vi "refresh Vbg.vi"(8 "stop":bool) -> (0 "X3":cluster{"Y":dbl[], "Y":dbl[]}[](graph), 1 "Zx 4":cluster{"Y":dbl[], "Y":dbl[]}[](graph), 2 "Zx 3":cluster{"Y":dbl[], "Y":dbl[]}[](graph), 3 "Temp vs Time":cluster{"Y":dbl[], "Y":dbl[]}[](graph), 4 "i X":cluster{"Y":dbl[], "Y":dbl[]}[](graph), 5 "X 2":cluster{"Y":dbl[], "Y":dbl[]}[](graph))   [LabVIEW 2011]
uses:
  DAQ-lockin-SubVI/Source/Lock-in Globles.vi
  SubVI/ITX_Global.vi
panel:
  in  "Tab Control":T1(tab)
  in  "Lock-in # 2":u16(ring)=1 items=["Lock-in #1", "Lock-in #2", "Lock-in #3", "Lock-in #4"]
  out "OSC Configuration":T2(array[cluster])=[{"Signal Type"=enum."Sine Wave", "DC"=0.0, "Amplitude"=0.15, "frequency"=1.3459999999999999, "Phase"=0.0}, {"Signal Type"=enum."Sine Wave", "DC"=0.0, "Amplitude"=0.0, "frequency"=1.346, "Phase"=0.0}, {"Signal Type"=enum."Sine Wave", "DC"=0.0, "Amplitude"=0.0, "frequency"=1.346, "Phase"=0.0}, {"Signal Type"=enum."Sine Wave", "DC"=0.0, "Amplitude"=0.0, "frequency"=1.346, "Phase"=0.0}] {"frequency" format="%0.2p"; "Amplitude" format="%0.2p"; "DC" format="%.2p"}
  in  "Lock-in # 1":u16(ring) items=["Lock-in #1", "Lock-in #2", "Lock-in #3", "Lock-in #4"]
  in  "Lock-in # 3":u16(ring)=2 items=["Lock-in #1", "Lock-in #2", "Lock-in #3", "Lock-in #4"]
  in  "Lock-in # 4":u16(ring)=3 items=["Lock-in #1", "Lock-in #2", "Lock-in #3", "Lock-in #4"]
  in  "milliseconds to wait":u32=1000
  in  "Comments":string="SA02628C 20120701\ncool down and warm up in ppms\n2 terminal tests.\nI+/I- : 3/27\nV+V-: 1/28\n\n\n\nno back gate voltage connected\n"
  out "Connected":string="I+:2\nV1+:3\nI-:28\nV-:5\n"
  in  "Vbg interval":u32=3000
  in  "Vo":dbl=-2.0
  in  "Vmax":dbl=7.0
  out "Vbg":dbl=-2.0
  in  "dV":dbl=0.01
  in  "Vmin":dbl=-2.0
  in  "OK Button":bool
  in  "Vsg     Vbg":bool
  in  "OSC config channel#":i32
  in  "Vsg interval":u32=3000
  out "Vsg":dbl
  out "Vbg vs time":cluster{"Y":dbl[], "Y":dbl[]}[](graph)
  out "Vsg vs time":cluster{"Y":dbl[], "Y":dbl[]}[](graph)
  out "i Y":cluster{"Y":dbl[], "Y":dbl[]}[](graph)
  out "i X 3":cluster{"Y":dbl[], "Y":dbl[]}[](graph)
  out "i Y 3":cluster{"Y":dbl[], "Y":dbl[]}[](graph)
  out "Y 2":cluster{"Y":dbl[], "Y":dbl[]}[](graph)
  out "Y3":cluster{"Y":dbl[], "Y":dbl[]}[](graph)
  out "Zy 3":cluster{"Y":dbl[], "Y":dbl[]}[](graph)
  out "Zy 4":cluster{"Y":dbl[], "Y":dbl[]}[](graph)
  out "i X 2":cluster{"Y":dbl[], "Y":dbl[]}[](graph)
  out "i X 4":cluster{"Y":dbl[], "Y":dbl[]}[](graph)
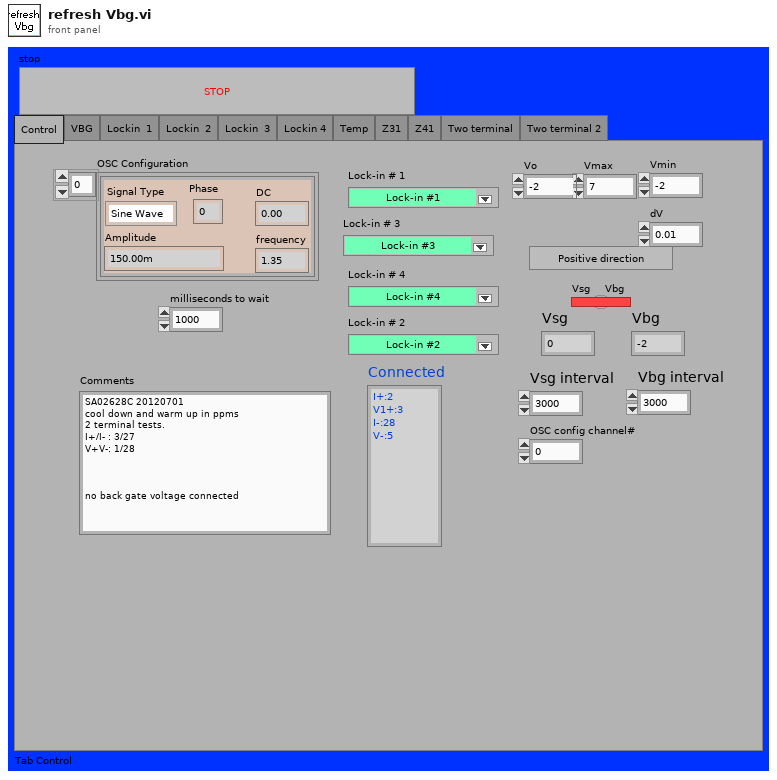
[diagram p1: front panel]
types:
  T1 = enum32{"Control", "VBG", "Lockin  1", "Lockin  2", "Lockin  3", "Lockin 4", "Temp", "Z31", "Z41", "Two terminal", "Two terminal 2"}
  T2 = cluster{"Signal Type":enum16{"Sine Wave", "Triangle Wave", "Square Wave", "Sawtooth Wave"}, "DC":dbl, "Amplitude":dbl, "frequency":dbl, "Phase":dbl}[]
  T3 = cluster{"Signal Type":enum16{"Sine Wave", "Triangle Wave", "Square Wave", "Sawtooth Wave"}, "DC":dbl, "Amplitude":dbl, "frequency":dbl, "Phase":dbl}
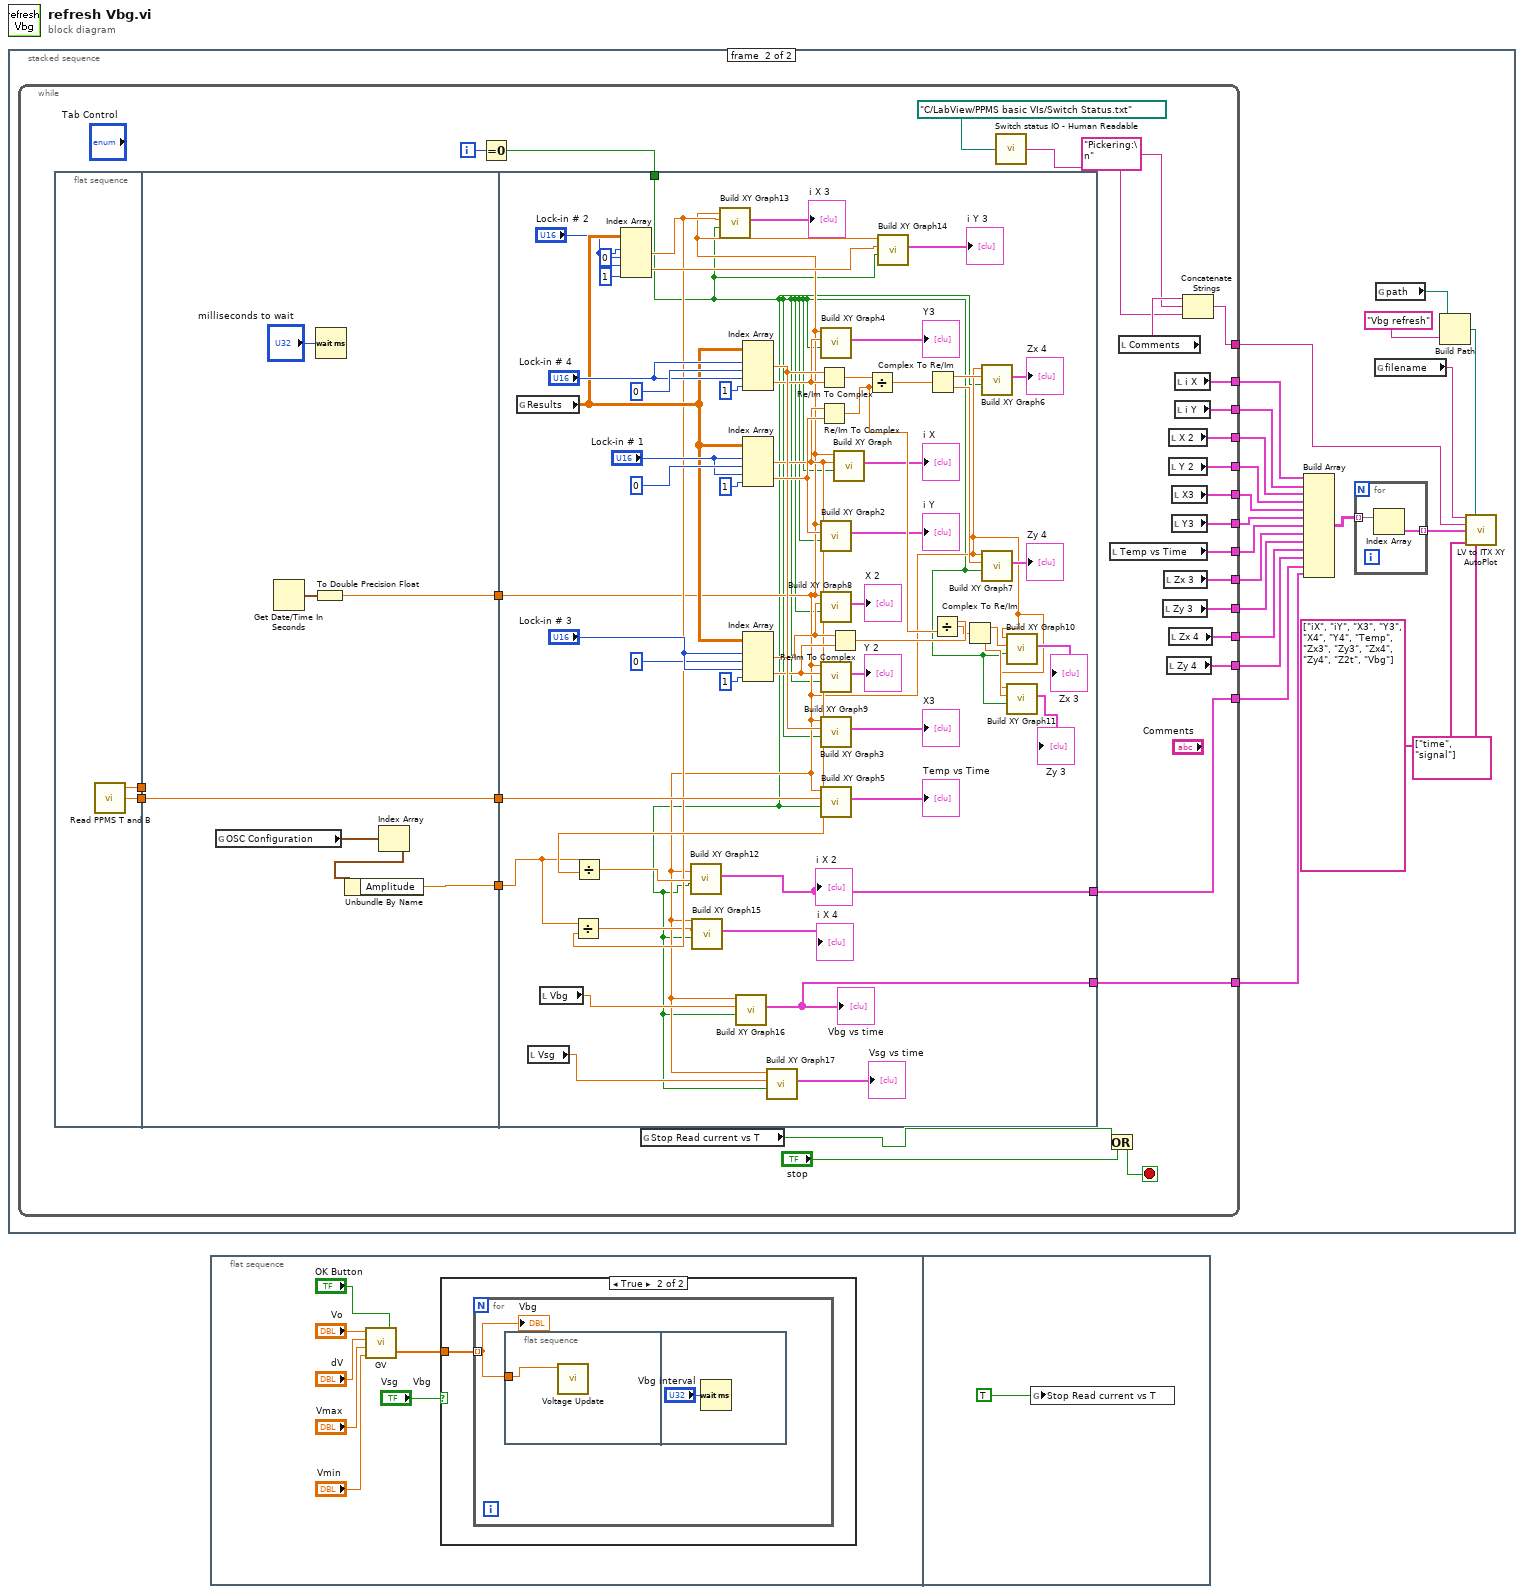
[diagram p0: block diagram]
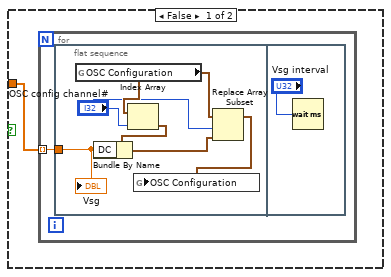
[diagram p2: hidden frame]
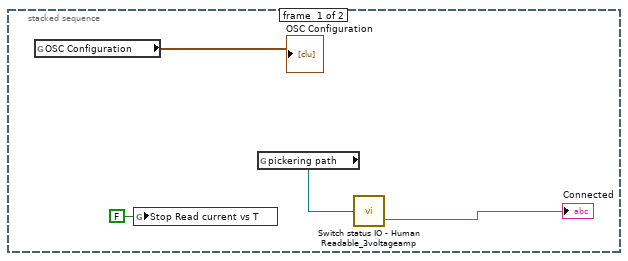
[diagram p3: hidden frame]
diagram:
  n1 = stacked-sequence {
    frame #0 {
      n2 = global read "Lock-in Globles.vi" "OSC Configuration"() -> (→"OSC Configuration":T2)
      n3 = global write "Lock-in Globles.vi" "Stop Read current vs T"(FALSE ("Stop Read current vs T")) -> ()
      n4 = global read "ITX_Global.vi" "pickering path"() -> (w1:path)
      n5 = call <userlib>:"Switch status IO - Human Readable_3voltageamp.vi"("Switch status"=w1) -> ("String"=→"Connected":string)  [unwired: 3 in]
    }
    frame #1 {
      n6 = while {
        tunnel: [w48] -> w26
        tunnel: [w47] -> w25
        tunnel: [w46] -> w24
        tunnel: [w45] -> w23
        tunnel: [w44] -> w22
        tunnel: [w43] -> w21
        tunnel: [w42] -> w20
        tunnel: [w41] -> w19
        tunnel: [w40] -> w18
        tunnel: [w39] -> w17
        tunnel: [w38] -> w16
        tunnel: [w36] -> w12
        tunnel: [w30] -> w6
        tunnel: [w29] -> w5
        i -> [w54]
        stop <- w50 stop-if-true
        n7 = flat-sequence {
          tunnel: [w58] -> w55
          tunnel: [w57] -> w51
          tunnel: [w64] -> w56
          tunnel: w55 -> [w64]
          tunnel: [w62] -> w52
          tunnel: w51 -> [_]
          tunnel: [w59] -> w31
          tunnel: w56 -> [w102]
          tunnel: w53 -> [w66]
          tunnel: w52 -> [w67]
          tunnel: w31 -> [w75]
          tunnel: [w83] -> w30
          tunnel: [w70] -> w29
          frame #0 {
            n8 = call "Read PPMS T and B.vi"() -> ("Temperature"=w58:dbl, "Time"=w57:dbl)  [unwired: 3 in, 1 out]
          }
          frame #1 {
            n9 = global read "Lock-in Globles.vi" "OSC Configuration"() -> (w61:T2)
            n10 = Get Date/Time In Seconds() -> (seconds since 1Jan1904=w63:timestamp)
            n11 = To Double Precision Float(number=w63) -> (double precision float=w62:dbl)
            n12 = Wait (ms)(milliseconds to wait="milliseconds to wait") -> ()  [unwired: 1 out]
            n13 = Index Array(array=w61) -> (element=w60:T3)  [unwired: 1 in]
            n14 = Unbundle By Name(w60) -> ("Amplitude"=w59:dbl)
          }
          frame #2 {
            n15 = global read "Lock-in Globles.vi" "Results"() -> (w82:dbl[][])
            n16 = local read "Vsg"() -> (w68:dbl)
            n17 = local read "Vbg"() -> (w71:dbl)
            n18 = Index Array(array=w82, index (row) #1="Lock-in # 2", index (col) #1=0 ("disabled index (col)"), index (row) #2="Lock-in # 2", index (col) #2=1 ("disabled index (col)")) -> (element #1=w74:dbl, element #2=w76:dbl)
            n19 = Divide(x=w75, y=w74) -> (x/y=w73:dbl)
            n20 = call "Build XY Graph15"("Reset"=w66, "Y Input"=w73, "X Input"=w67) -> ("XY Graph"=→"i X 4":cluster{"Y":dbl[], "Y":dbl[]}[])  [unwired: 2 in, 6 out]
            n21 = call "Build XY Graph13"("Reset"=w66, "Y Input"=w74, "X Input"=w67) -> ("XY Graph"=→"i X 3":cluster{"Y":dbl[], "Y":dbl[]}[])  [unwired: 2 in, 6 out]
            n22 = call "Build XY Graph16"("Reset"=w66, "Y Input"=w71, "X Input"=w67) -> ("XY Graph"=w70:cluster{"Y":dbl[], "Y":dbl[]}[])  [unwired: 2 in, 6 out]
            "Vbg vs time" <- w70
            n23 = Index Array(array=w82, index (row) #1="Lock-in # 4", index (col) #1=0 ("disabled index (col)"), index (row) #2="Lock-in # 4", index (col) #2=1 ("disabled index (col)")) -> (element #1=w110:dbl, element #2=w109:dbl)
            n24 = Index Array(array=w82, index (row) #1="Lock-in # 1", index (col) #1=0 ("disabled index (col)"), index (row) #2="Lock-in # 1", index (col) #2=1 ("disabled index (col)")) -> (element #1=w85:dbl, element #2=w111:dbl)
            n25 = Divide(x=w75, y=w85) -> (x/y=w84:dbl)
            n26 = call "Build XY Graph12"("Reset"=w66, "Y Input"=w84, "X Input"=w67) -> ("XY Graph"=w83:cluster{"Y":dbl[], "Y":dbl[]}[])  [unwired: 2 in, 6 out]
            "i X 2" <- w83
            n27 = Index Array(array=w82, index (row) #1="Lock-in # 3", index (col) #1=0 ("disabled index (col)"), index (row) #2="Lock-in # 3", index (col) #2=1 ("disabled index (col)")) -> (element #1=w96:dbl, element #2=w95:dbl)
            n28 = call "Build XY Graph17"("Reset"=w66, "Y Input"=w68, "X Input"=w67) -> ("XY Graph"=→"Vsg vs time":cluster{"Y":dbl[], "Y":dbl[]}[])  [unwired: 2 in, 6 out]
            n29 = Re/Im To Complex(1:w109, 2:w110) -> (0:w108:cdb)
            n30 = Re/Im To Complex(1:w111, 2:w85) -> (0:w93:cdb)
            n31 = call "Build XY Graph4"("Reset"=w66, "Y Input"=w109, "X Input"=w67) -> ("XY Graph"=→"Y3":cluster{"Y":dbl[], "Y":dbl[]}[])  [unwired: 2 in, 6 out]
            n32 = call "Build XY Graph2"("Reset"=w66, "Y Input"=w111, "X Input"=w67) -> ("XY Graph"=→"i Y":cluster{"Y":dbl[], "Y":dbl[]}[])  [unwired: 2 in, 6 out]
            n33 = call "Build XY Graph8"("Reset"=w66, "Y Input"=w96, "X Input"=w67) -> ("XY Graph"=→"X 2":cluster{"Y":dbl[], "Y":dbl[]}[])  [unwired: 2 in, 6 out]
            n34 = call "Build XY Graph9"("Reset"=w66, "Y Input"=w95, "X Input"=w67) -> ("XY Graph"=→"Y 2":cluster{"Y":dbl[], "Y":dbl[]}[])  [unwired: 2 in, 6 out]
            n35 = call "Build XY Graph3"("Reset"=w66, "Y Input"=w110, "X Input"=w67) -> ("XY Graph"=→"X3":cluster{"Y":dbl[], "Y":dbl[]}[])  [unwired: 2 in, 6 out]
            n36 = call "Build XY Graph5"("Reset"=w66, "Y Input"=w102, "X Input"=w67) -> ("XY Graph"=→"Temp vs Time":cluster{"Y":dbl[], "Y":dbl[]}[])  [unwired: 2 in, 6 out]
            n37 = Re/Im To Complex(1:w95, 2:w96) -> (0:w94:cdb)
            n38 = call "Build XY Graph"("Reset"=w66, "Y Input"=w85, "X Input"=w67) -> ("XY Graph"=→"i X":cluster{"Y":dbl[], "Y":dbl[]}[])  [unwired: 2 in, 6 out]
            n39 = Divide(x=w108, y=w93) -> (x/y=w107:cdb)
            n40 = call "Build XY Graph14"("Reset"=w66, "Y Input"=w76, "X Input"=w67) -> ("XY Graph"=→"i Y 3":cluster{"Y":dbl[], "Y":dbl[]}[])  [unwired: 2 in, 6 out]
            n41 = Complex To Re/Im(x + iy=w107) -> (x=w105:dbl, y=w106:dbl)
            n42 = Divide(x=w94, y=w93) -> (x/y=w92:cdb)
            n43 = Complex To Re/Im(x + iy=w92) -> (x=w91:dbl, y=w90:dbl)
            n44 = call "Build XY Graph6"("Reset"=w66, "Y Input"=w105, "X Input"=w67) -> ("XY Graph"=→"Zx 4":cluster{"Y":dbl[], "Y":dbl[]}[])  [unwired: 2 in, 6 out]
            n45 = call "Build XY Graph7"("Reset"=w66, "Y Input"=w106, "X Input"=w67) -> ("XY Graph"=→"Zy 4":cluster{"Y":dbl[], "Y":dbl[]}[])  [unwired: 2 in, 6 out]
            n46 = call "Build XY Graph10"("Reset"=w66, "Y Input"=w91, "X Input"=w67) -> ("XY Graph"=→"Zx 3":cluster{"Y":dbl[], "Y":dbl[]}[])  [unwired: 2 in, 6 out]
            n47 = call "Build XY Graph11"("Reset"=w66, "Y Input"=w90, "X Input"=w67) -> ("XY Graph"=→"Zy 3":cluster{"Y":dbl[], "Y":dbl[]}[])  [unwired: 2 in, 6 out]
          }
        }
        n48 = Equal To 0?(x=w54) -> (x = 0?=w53:bool)
        n49 = global read "Lock-in Globles.vi" "Stop Read current vs T"() -> (w32:bool)
        n50 = call <userlib>:"Switch status IO - Human Readable.vi"("Switch status"=path "C:/LabView/PPMS basic VIs/Switch Status.txt") -> ("String"=w33:string)
        n51 = Or(x=w32, y="stop") -> (x .or. y?=w50:bool)
        n52 = local read "Temp vs Time"() -> (w42:cluster{"Y":dbl[], "Y":dbl[]}[])
        n53 = local read "Comments"() -> (w35:string)
        n54 = local read "Zy 3"() -> (w40:cluster{"Y":dbl[], "Y":dbl[]}[])
        n55 = local read "Zx 3"() -> (w41:cluster{"Y":dbl[], "Y":dbl[]}[])
        n56 = local read "Zy 4"() -> (w38:cluster{"Y":dbl[], "Y":dbl[]}[])
        n57 = local read "X 2"() -> (w46:cluster{"Y":dbl[], "Y":dbl[]}[])
        n58 = local read "Y 2"() -> (w45:cluster{"Y":dbl[], "Y":dbl[]}[])
        n59 = local read "Zx 4"() -> (w39:cluster{"Y":dbl[], "Y":dbl[]}[])
        n60 = local read "X3"() -> (w44:cluster{"Y":dbl[], "Y":dbl[]}[])
        n61 = local read "Y3"() -> (w43:cluster{"Y":dbl[], "Y":dbl[]}[])
        n62 = local read "i X"() -> (w48:cluster{"Y":dbl[], "Y":dbl[]}[])
        n63 = local read "i Y"() -> (w47:cluster{"Y":dbl[], "Y":dbl[]}[])
        n64 = Concatenate Strings(w35, "Pickering:\n" ("string"), w33) -> (w36:string)
      }
      n65 = Build Array(w26, w25, w24, w23, w22, w21, w20, w19, w18, w17, w16, w6, w5) -> (w15:cluster{"Y":dbl[], "Y":dbl[]}[][])
      n66 = for {
        tunnel: w15 -> [w28] mode=indexing
        tunnel: [w27] -> w14 mode=indexing
        n67 = Index Array(array=w28) -> (element=w27:cluster{"Y":dbl[], "Y":dbl[]})  [unwired: 1 in]
      }
      n68 = global read "ITX_Global.vi" "filename"() -> (w13:string)
      n69 = global read "ITX_Global.vi" "path"() -> (w9:path)
      n70 = Build Path(base path=w9, name or relative path="Vbg refresh") -> (appended path=w8:path)
      n71 = call <userlib>:"LV to ITX XY AutoPlot.vi"("filename"=w13, "path"=w8, "Notes"=w12, "XY Array"=w14, "wavenames (.Vx, etc)"=string[] ["iX", "iY", "X3", "Y3", "X4", "Y4", "Temp", "Zx3", "Zy3", "Zx4", "Zy4", "Z2t", "Vbg"], "X,Y Labels"=string[] ["time", "signal"]) -> ()  [unwired: 9 in, 1 out]
    }
  }
  n72 = flat-sequence {
    frame #0 {
      n73 = call "GV.vi"("OK Button"="OK Button", "Vmin"="Vmin", "Vmax"="Vmax", "dV"="dV", "Vo"="Vo") -> ("Waveform Graph"=w122:dbl[])
      n74 = case shown="True" "Vsg     Vbg" {
        tunnel: w122 -> [w128 w137]
        frame False {
          n75 = for {
            tunnel: w128 -> [w129] mode=indexing
            n76 = flat-sequence {
              tunnel: w129 -> [w130]
              frame #0 {
                n77 = global read "Lock-in Globles.vi" "OSC Configuration"() -> (w134:T2)
                n78 = Index Array(array=w134, index="OSC config channel#") -> (element=w135:T3)
                n79 = Bundle By Name(cluster=w135, "DC"=w130) -> (w132:T3)
                n80 = Replace Array Subset(array=w134, new element=w132, index="OSC config channel#") -> (w131:T2)
                n81 = global write "Lock-in Globles.vi" "OSC Configuration"(w131) -> ()
                "Vsg" <- w130
              }
              frame #1 {
                n82 = Wait (ms)(milliseconds to wait="Vsg interval") -> ()  [unwired: 1 out]
              }
            }
          }
        }
        frame True {
          n83 = for {
            tunnel: w137 -> [w138] mode=indexing
            n84 = flat-sequence {
              tunnel: w138 -> [w139]
              frame #0 {
                n85 = call "Voltage Update.vi"("Voltage Output"=w139) -> ()  [unwired: 8 in]
              }
              frame #1 {
                n86 = Wait (ms)(milliseconds to wait="Vbg interval") -> ()  [unwired: 1 out]
              }
            }
            "Vbg" <- w138
          }
        }
      }
    }
    frame #1 {
      n87 = global write "Lock-in Globles.vi" "Stop Read current vs T"(TRUE ("Stop Read current vs T")) -> ()
    }
  }
